vi "TDMSWrite(SubVI)_6ch.vi"(0 "tdms file out 입력":refnum<k34>, 1 "배열":dbl[](array[numeric]), 5 "그룹입력":string="Robot-M1509", 7 "채널입력":string[](array[string]), 11 "에러 입력":errorcluster caption="에러 입력(에러 없음)") -> (4 "참조 번호 출력":refnum<k34>, 15 "에러 출력":errorcluster)   [LabVIEW 2019]
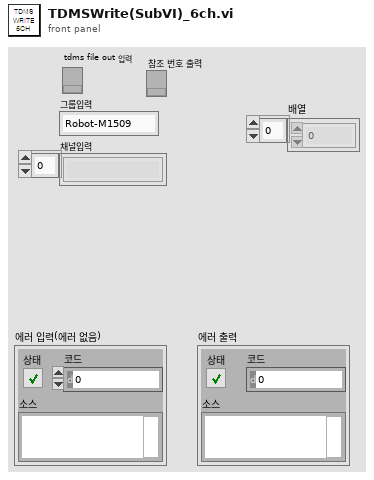
[diagram p1: front panel]
types:
  T1 = cluster{"배열[0]":dbl, "배열[1]":dbl, "배열[2]":dbl, "배열[3]":dbl, "배열[4]":dbl, "배열[5]":dbl, "배열[6]":dbl, "배열[7]":dbl, "배열[8]":dbl}
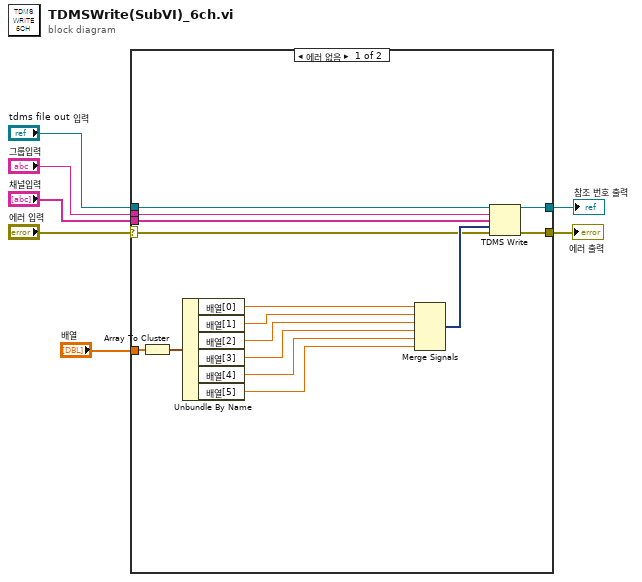
[diagram p0: block diagram]
diagram:
  n1 = case shown="에러 없음" "에러 입력" {
    selector: "에러 입력" -> [w18 w23]
    tunnel: [w21 w24] -> w7
    tunnel: [w20 w23] -> w6
    tunnel: "tdms file out 입력" -> [w19 w24]
    tunnel: "그룹입력" -> [w17 _]
    tunnel: "채널입력" -> [w16 _]
    tunnel: "배열" -> [w15 _]
    frame No Error {
      n2 = Array To Cluster(array=w15) -> (cluster=w14:T1)
      n3 = Unbundle By Name(w14) -> ("배열[0]"=w13:dbl, "배열[1]"=w12:dbl, "배열[2]"=w11:dbl, "배열[3]"=w10:dbl, "배열[4]"=w9:dbl, "배열[5]"=w8:dbl)
      n4 = Merge Signals(w13, w12, w11, w10, w9, w8) -> (w22:dynamicdata)
      n5 = TDMS Write(0:w19, 5:w17, 7:w16, 9:w22, 11:w18) -> (4:w21:refnum<k34>, 15:w20:errorcluster)  [unwired: 1 in, 2 out]
    }
    frame Error {
    }
  }
  "참조 번호 출력" <- w7
  "에러 출력" <- w6
